vi "SC Get Project.vi"(8 "error in (no error)":errorcluster) -> (0 "error out":errorcluster, 1 "project folder":path, 2 "found?":bool, 3 "project application":refnum<vi>)   [LabVIEW 2023]
doc: "The folder of the project the Tools menu was used from: the project of the VI window whose menu launched this tool (Application:Menu Launch:App, readable once per launch, so this is called once, at the start), else LabVIEW's active project (a Project Explorer window's menu, or no menu launch). If no project is open, tells the user to open one and returns found? = false."
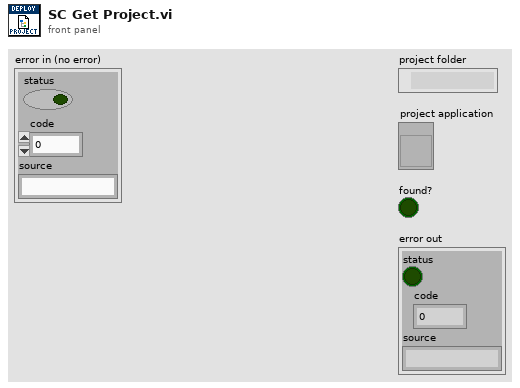
[diagram p1: front panel]
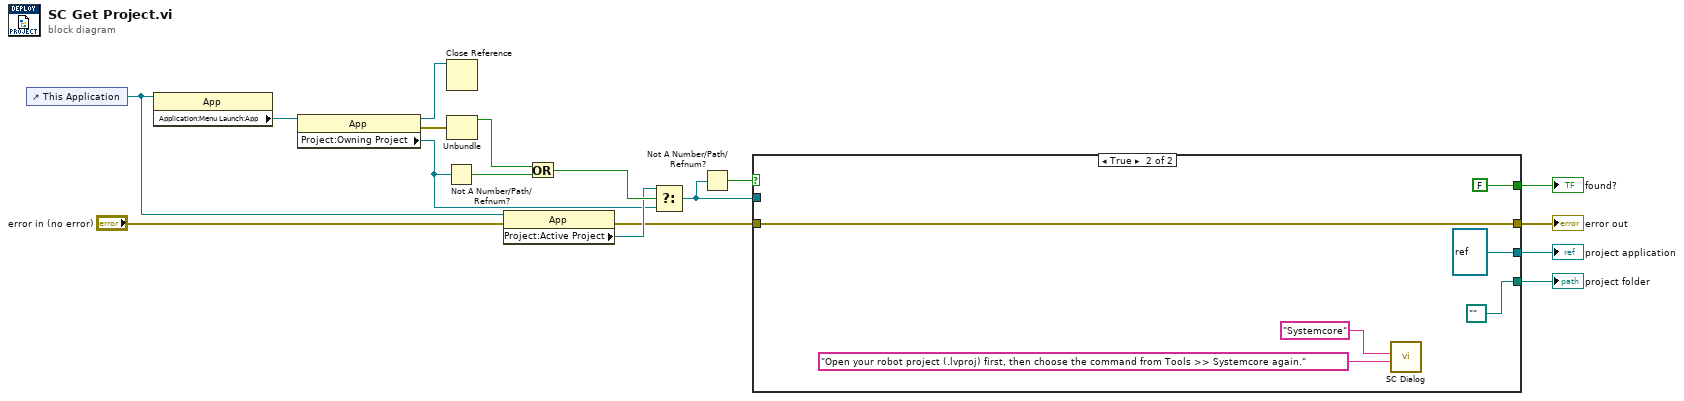
[diagram p0: block diagram]
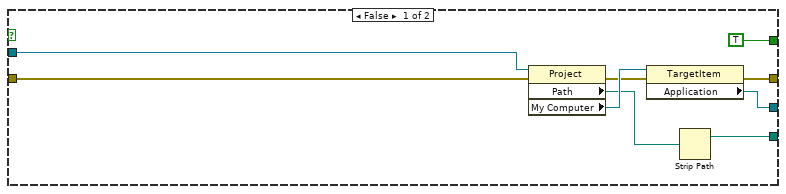
[diagram p2: hidden frame]
diagram:
  n1 = control-ref of="This Application"() -> (w12:refnum<vi>)
  n2 = property class="App"(reference=w12) -> ("Application:Menu Launch:App"=w17:refnum<vi>)  [unwired: 1 in, 2 out]
  n3 = property class="App"(reference=w17) -> (reference out=w16:refnum<vi>, error out=w15:errorcluster, "Project:Owning Project"=w8:refnum<vi>)  [unwired: 1 in]
  n4 = Not A Number/Path/Refnum?(number/path/refnum=w8) -> (NaN/Path/Refnum?=w13:bool)
  n5 = Close Reference(reference=w16) -> ()  [unwired: 1 in, 1 out]
  n6 = Unbundle(w15) -> ("status"=w14:bool)  [unwired: 2 out]
  n7 = property class="App"(reference=w12, error in="error in (no error)") -> (error out=w6:errorcluster, "Project:Active Project"=w9:refnum<vi>)  [unwired: 1 out]
  n8 = Or(x=w14, y=w13) -> (x .or. y?=w10:bool)
  n9 = Select(t=w9, s=w10, f=w8) -> (s? t:f=w7:refnum<vi>)
  n10 = Not A Number/Path/Refnum?(number/path/refnum=w7) -> (NaN/Path/Refnum?=w1:bool)
  n11 = case shown="True" w1 {
    tunnel: w7 -> [w26 _]
    tunnel: w6 -> [w25 w28]
    tunnel: [w20 path ""] -> w5
    tunnel: [TRUE FALSE] -> w4
    tunnel: [w18 w28] -> w3
    tunnel: [w22 refnum<vi> refnum] -> w2
    frame False {
      n12 = property class="Project"(reference=w26, error in=w25) -> (error out=w23:errorcluster, "Path"=w21:path, "My Computer"=w24:refnum<vi>)  [unwired: 1 out]
      n13 = property class="TargetItem"(reference=w24, error in=w23) -> (error out=w18:errorcluster, "Application"=w22:refnum<vi>)  [unwired: 1 out]
      n14 = Strip Path(path=w21) -> (stripped path=w20:path)  [unwired: 1 out]
    }
    frame True {
      n15 = call "SC Dialog.vi"("message"="Open your robot project (.lvproj) first, then choose the command from Tools >> Systemcore again.", "window title"="Systemcore") -> ()  [unwired: 9 in, 1 out]
    }
  }
  "project folder" <- w5
  "project application" <- w2
  "found?" <- w4
  "error out" <- w3
